vi "AlliGator Image Histogram Panel.vi"() -> ()   [LabVIEW 2021, in "AlliGator Image Histogram.lvlib"]
uses:
  AlliGator Image Histogram.lvlib
  Histograms/Linear Histogram Options.ctl
  Histograms/Histogram Bin Option.ctl
  Histograms/Histogram Bin Position.ctl
  AlliGator Image Histogram Control Refnums.ctl
  Globals, Variables, Constants/AlliGator Refnums List.ctl
  Settings/AlliGator Settings List.ctl
  Action Engine/AlliGator Q Element.ctl
  Action Engine/AlliGator Q Event.ctl
  Source Image/AlliGator Dataset Ctrl Refnums.ctl
  Utilities/Read-Write.ctl
  Graphs/XY Graph/XY Graph Event.ctl
  <vilib>/Utility/miscctls.llb/LVPoint32TypeDef.ctl
  Variant/Variant to Data/Variant to Boolean.vi
  Settings/AlliGator Settings+.lvlib
  Variant/Variant to Data/Variant to Data.lvlib
  Notebook/Notebook.lvlib
  Action Engine/AlliGator Action Engine.lvlib
  Graphs/XY Graph/XY Graph Add-Ons.lvlib
  Python Plugins API/AlliGator Python Plugins.lvlib
  GUI/AlliGator GUI.lvlib
  Utilities/Utilities.lvlib
  GUI/GUI.lvlib
  Error/Error.lvlib
  Histograms/Histograms.lvlib
panel:
  in  "Pin Button":bool=TRUE
  in  "Histogram Lower Percentile":dbl=1.0 caption="Lower Percentile" min=0.0 max=100.0 format="%#.3f"
  in  "Histogram Upper Percentile":dbl=1.0 caption="100 - Upper Percentile" min=0.0 max=100.0 format="%#.3f"
  in  "Auto-Adjust Contrast":bool=TRUE
  in  "Image Histogram Active":bool=TRUE
  in  "Use Image Histogram for Contrast":bool=TRUE
  out "Image Histogram":cluster{"X Array":dbl[], "Y Array":dbl[]}[](graph)
  in  "Image Histogram Options":T1={"Bin Size"=1.0, "Bin Number"=256, "Bin Option"=enum."Bin Number", "Min Value"=-inf, "Max Value"=inf, "Filter NaN & Infinite Values"=TRUE, "Frequency Plot"=FALSE, "Align Bins"=TRUE, "Bin Location"=enum."Left", "Project Outside Values"=FALSE, "Max Histogram Size"=1000000} {"Max Histogram Size" format="%.0e"}
  out "Lower Percentile":dbl=nan format="%#_5g"
  out "Upper Percentile":dbl=nan format="%#_5g"
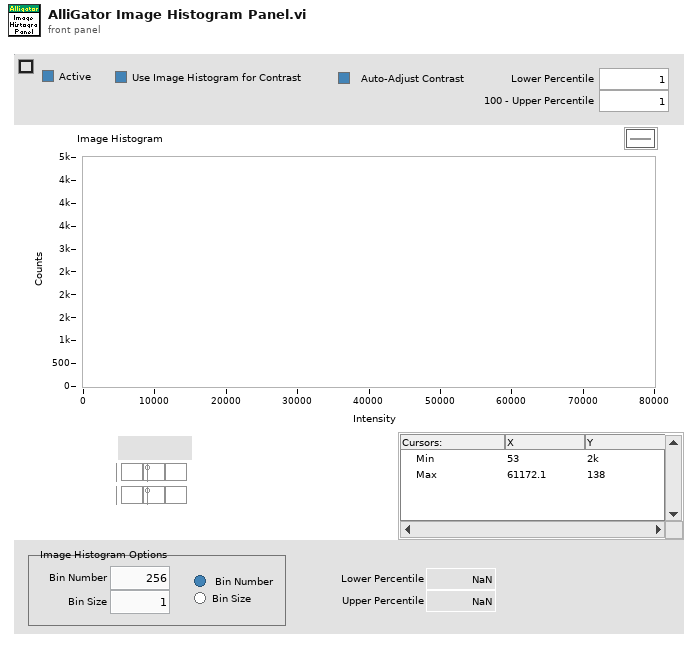
[diagram p1: front panel]
types:
  T1 = typedef "Histograms.lvlib/Linear Histogram Options.ctl" = cluster{"Bin Size":dbl, "Bin Number":i32, "Bin Option":T2, "Min Value":dbl, "Max Value":dbl, "Filter NaN & Infinite Values":bool, "Frequency Plot":bool, "Align Bins":bool, "Bin Location":T3, "Project Outside Values":bool, "Max Histogram Size":i32}
  T2 = typedef "Histograms.lvlib/Histogram Bin Option.ctl" = enum32{"Bin Number", "Bin Size"}
  T3 = typedef "Histograms.lvlib/Histogram Bin Position.ctl" = enum16{"Left", "Center", "Right"}
  T4 = typedef "AlliGator GUI.lvlib/AlliGator Refnums List.ctl" = enum16{"---------- AlliGator Control Refnums ----------", "AlliGator Tab Control Refnum", "Dataset Ctrl Refnums", "Image Histogram Ctrl Refnums", "Intensity Time Trace Ctrl Refnums", "Decay Graph Ctrl Refnums", "Decay Statistics Graph Ctrl Refnums", "Phasor Graph Ctrl Refnums", "Phasor Ratio Graph Ctrl Refnums", "Phasor Plot Ctrl Refnums", "Lifetime & Other Parameters Ctrl Refnums", "Decay Fit Parameter Map Ctrl Refnums", "Parameter Map Ctrl Refnums", "Other AlliGator Ctrl Refnums", "---------- AlliGator Menu Refnums ----------", "AlliGator Menu", "---------- IO Device ID ----------", "Mouse ID", "Keyboard ID"}
  T5 = typedef "AlliGator Image Histogram.lvlib/AlliGator Image Histogram Control Refnums.ctl" = cluster{"Image Histogram":refnum<vi>, "Image Histogram Options":refnum<vi>, "Image Histogram Active":refnum<vi>, "Image Histogram Upper Percentile":refnum<vi>, "Image Histogram Lower Percentile":refnum<vi>, "Auto-Adjust Contrast":refnum<vi>}
  T6 = typedef "AlliGator Settings+.lvlib/AlliGator Settings List.ctl" = enum16{"GUI:Visible Settings Tab", "GUI:Last Run Version", "Source Image:Use Image Histogram for Contrast", "Source Image:Low Count Pixels Rejection Options", "Source Image:High Count Pixels Rejection Options", "Source Image:Use Image Brightness", "Source Image:Blend Overlay with Image Background", "Source Image:Use Fixed ROI Diameter", "Source Image:ROI Diameter", "Source Image:ROI Center Color", "Source Image:Peak Threshold", "Source Image:Intensity Threshold", "Source Image:Image Binning Options", "Source Image:Image Smoothing Options", "Source Image:Image Histogram Active", "Source Image:Invert Binary Mask", "Source Image:Hot Pixel Removal", "Source Image:Overlay Analyzed ROI Center", "Source Image:Auto-Adjust Contrast", "Source Image:Histogram Lower Percentile", "Source Image:Histogram Upper Percentile", "Source Image:Lock ROI with Maps", "Source Image:Save Source Image", "Source Image:Scale Bar Options", "Source Image:Image Resolution (Pixel Size)", "Source Image:Flatfield Correction", "Source Image:Show Dead Left Columns Correction", "Source Image:Dead Left Columns Correction", "Source Image:Image Pre-Processing Operations Order", "Source Image:Overlay ROI Median", "Source Image:Median Overlay Color", "Data Information:Gate Width", "Data Information:Nanotime Gate Separation", "Data Information:Macrotime Gate Separation", "Data Information:Gate Step", "Data Information:# Gates", "Data Information:Gate Image Exposure", "Data Information:Gate Image Integration", "Data Information:Gates to Skip", "Data Information:Gates to Keep", "Data Information:Define Gates to", "Data Information:Channel Name", "Data Information:Available Channel Names", "Data Information:Channel Arithmetic", "Data Information:Background File Subtraction", "Data Information:Background File", "Data Information:Background Scaling Factor", "Data Information:Background Pile-up Correction", "Data Information:Background Pixel Well Capacity", "Data Information:Laser Period", "Data Information:SYNC Period", "Data Information:Pile-up Correction", "Data Information:Pixel Well Capacity", "Data Information:Dataset Scaling Factor", "Fluorescence Decay_Decay Pre-Processing:Reverse Gates", "Fluorescence Decay_Decay Pre-Processing:Verbose Decay Pre-Processing", "Fluorescence Decay_Decay Pre-Processing:Use Decay Pre-Processing", "Fluorescence Decay_Decay Pre-Processing:Background Subtraction", "Fluorescence Decay_Decay Pre-Processing:Background Definition Range", "Fluorescence Decay_Decay Pre-Processing:Baseline Subtraction Method", "Fluorescence Decay_Decay Pre-Processing:Decay Pre-Processing Operations Order", "Fluorescence Decay_Decay Pre-Processing:Smoothing Parameter", "Fluorescence Decay_Decay Pre-Processing:Shift Decay", "Fluorescence Decay_Decay Pre-Processing:Decay Shift Parameters", "Fluorescence Decay_Decay Pre-Processing:Fold Decay", "Fluorescence Decay_Decay Pre-Processing:# Folds", "Fluorescence Decay_Decay Pre-Processing:1-Normalize Decay", "Fluorescence Decay_Decay Pre-Processing:[0-1]-Normalize Decay", "Fluorescence Decay_Decay Pre-Processing:Smoothen Decay", "Fluorescence Decay_Decay Pre-Processing:Extrapolate Decay", "Fluorescence Decay_Decay Pre-Processing:Use Periodicity", "Fluorescence Decay_Decay Pre-Processing:Use Cursors", "Fluorescence Decay_Decay Pre-Processing:Tail Fraction", "Fluorescence Decay_Decay Pre-Processing:Head Fraction", "Fluorescence Decay_Decay Pre-Processing:Additional Points", "Fluorescence Decay_Decay Pre-Processing:Straighten Decay", "Fluorescence Decay_Decay Pre-Processing:Constant Background", "Fluorescence Decay_Decay Pre-Processing:Pixel-Normalize Decay", "Fluorescence Decay_Advanced Analysis:Extract IRF instead of Decay", "Fluorescence Decay_Advanced Analysis:IRF Extraction Options", "Fluorescence Decay_Advanced Analysis:IRF Optimization Options", "Fluorescence Decay_Advanced Analysis:Square Pulse Options", "Fluorescence Decay_Advanced Analysis:IRF Order", "Fluorescence Decay_Advanced Analysis:IRF Time Constants", "Fluorescence Decay_Advanced Analysis:Wavelet Analysis Options", "Fluorescence Decay_Advanced Analysis:Average Lifetime Options", "Fluorescence Decay_Fit Options:Fit Options", "Fluorescence Decay_Fit Options:Use Legacy Fitting Approach", "Fluorescence Decay_Fit Options:Use Data Information Laser Period", "Fluorescence Decay_Fit Parameters:Displayed Fit Parameters", "Fluorescence Decay_Fit Parameters:Fit Parameter Constraints", "Fluorescence Decay_Fit Parameters:Export Tabulated Results", "Fluorescence Decay_Fit Parameters:MLE Baseline Offset Type", "Fluorescence Decay_Fit Parameters:MLE Baseline Offset", "Fluorescence Decay_Fit Parameters:Guess Parameter Names", "Fluorescence Decay_Fit Parameters:Guess Parameter Values", "Fluorescence Decay_Fit Parameters:Guess Parameters Options", "Fluorescence Decay_Fit Parameters:Optimal Offset Selection Criterion", "Fluorescence Decay_Styles:Show Last Decay Only", "Fluorescence Decay_Styles:Decay Graph Color Array", "Fluorescence Decay:Decay Graph Active", "Fluorescence Decay Statistics:Min Peak Value", "Fluorescence Decay Statistics:Reject Low Decay Peak Pixels", "Fluorescence Decay Statistics:Reject High Decay Peak Pixels", "Fluorescence Decay Statistics:Max Peak Value", "Time Traces:Use File Timestamp", "Time Traces:Time Step", "Time Traces:Use Intensity Correction File", "Time Traces:Intensity Correction File", "Phasor Plot:Phasor Plot Smoothing Options", "Phasor Plot:Phasor Plot Size", "Phasor Plot:Phasor Plot Graphics Options", "Phasor Plot:Cumulative Phasor Plot", "Phasor Plot:Use Phasor Brightness", "Phasor Plot:Blend Overlay with Phasor Background", "Phasor Plot:Save Phasor Plot", "Phasor Plot:Show References", "Phasor Plot:Phasor Ratio Decay Range", "Phasor Plot:Exponential Fading", "Phasor Plot:Phasor Ratio Reference Colors", "Phasor Plot:Reference Radius", "Phasor Plot:Show Color Map Vertices", "Phasor Plot:Phasor Plot Active", "Phasor Plot:Phasor Ratio Color Map Type", "Phasor Plot:Phasor Ratio Color Map", "Phasor Plot:Phasor Ratio Display Range", "Phasor Plot:Selected Image ROI(s)", "Phasor Plot:All Image ROIs", "Phasor Plot:Selected Phasor Plot ROI(s)", "Phasor Plot:All Phasor Plot ROIs", "Phasor Plot:Phasor Ratio Color-Coded Quantity", "Phasor Plot:Store Phasor Harmonics", "Phasor Plot:Draw Reference Segment", "Phasor Plot:User-Defined Quantity", "Phasor Plot:Color Scale High Color", "Phasor Plot:Color Scale Low Color", "Phasor Plot:Intensity-weighted Phasor Plot", "Phasor Graph:Phasor Frequency", "Phasor Graph:Phasor Ratio Type", "Phasor Graph:Pixel-level Phasor Computation", "Phasor Graph:Save Phasor Graph", "Phasor Graph:Phasor Graph Active", "Phasor Graph:Phasor SDV Options", "Phasor Graph:Intensity-weighted Phasor Graph", "Phasor Graph:Define Shortest Lifetime as", "Phasor Calibration:Use Backup Calibration if needed", "Phasor Calibration:Backup Calibration Type", "Phasor Calibration:Calibration Type", "Phasor Calibration:Calibration Lifetime", "Phasor Calibration:Calibration Map Algorithm", "Single-Exponential Phasor Locus (SEPL):Gate Parameters", "Single-Exponential Phasor Locus (SEPL):User-defined Gate", "Single-Exponential Phasor Locus (SEPL):User-defined IRF", "Single-Exponential Phasor Locus (SEPL):Phasor Parameters", "Single-Exponential Phasor Locus (SEPL):Decay & IRF Parameters", "Single-Exponential Phasor Locus (SEPL):Display Parameters", "Lifetime Analysis:Decay Analysis Parameters", "Lifetime Analysis:Lifetime Map Active", "Plugins:Python Settings", "Miscellaneous:Verbose Mode", "Miscellaneous:Beep after Script", "Miscellaneous:Saved Image File Format", "Miscellaneous:Exported Gate Image Settings", "Miscellaneous:Include Loading in Timing", "Miscellaneous:Verbose Settings Mode", "Miscellaneous:Histogram Options", "Miscellaneous:Beep on Error", "Miscellaneous:# Logical Processors Used", "Miscellaneous:ROI Description Max Characters", "Miscellaneous:Verbose Error Mode", "Miscellaneous:Transparent Mask Color"}
  T7 = typedef "AlliGator Action Engine.lvlib/AlliGator Q Element.ctl" = cluster{"AlliGator Q Event":T8, "Data":variant}
  T8 = typedef "AlliGator Action Engine.lvlib/AlliGator Q Event.ctl" = enum16{"---- Files ----", "Files:Set Batch Export Files To Save", "Files:Set Dataset Loading & Pre-processing Options", "Files:Check #Frames in Dataset", "Files:Increment Frame Index", "Files:Open Mask Image", "Files:Open White Light Image", "Files:Open Single Dataset", "Files:New Folder of Folders Selected", "Files:Load File (all Types)_Scriptable", "Files:Move Flattened Series to Folders Series", "Files:Select Folder", "Files:Load FLI Dataset", "Files:Load Swiss SPAD 1 Dataset", "Files:Load Swiss SPAD 2 Dataset", "Files:Load .sdt FLI Dataset", "Files:Load .ptu FLI Dataset", "Files:Load .bin FLI Dataset", "Files:Load Single Gate Image Folder", "Files:Load I/m/phi Dataset (deprecated)", "Files:Load Single Image", "Files:Subtract Background File", "Files:Export FLI Dataset", "Files:Load HDF5 FLI Dataset", "Files:Set Destination File Path", "Files:Save Mask Image", "Files:Batch Conversion", "Files:New Folder Selected", "Files:Close FLI Dataset", "Files:Close FLI Dataset Series", "Files:Close White Light Image", "Files:Close Mask Image", "---- FLI Dataset ----", "FLI Dataset:Channel Arithmetic", "FLI Dataset:Export Average Lifetime Map as ASCII", "FLI Dataset:Export User-Defined Quantity Map as ASCII", "FLI Dataset:Python Function FLI Dataset Event", "FLI Dataset:ROI Analysis", "FLI Dataset:Tilted Logistic Square Gated IRF Characteristics Map", "FLI Dataset:Logistic Square Gated IRF Characteristics Map", "FLI Dataset:Square Gated IRF Characteristics Map", "FLI Dataset:Multi-ROI Single-Pixel Phasor Analysis", "FLI Dataset:Multi-ROI Single-Pixel NLSF Analysis", "FLI Dataset:All ROIs IRF Extraction", "FLI Dataset:All ROIs Decay Fit Non-Interactive (Fast + Individual IRF)", "FLI Dataset:All ROIs Phasor Analysis", "FLI Dataset:All ROIs Decay Fit", "FLI Dataset:Fluorescence Decay Statistics", "FLI Dataset:Update Decay Statistics Graph", "FLI Dataset:Get Decay from ROI", "FLI Dataset:All ROIs Average Lifetimes", "FLI Dataset:Save/Load Local IRFs", "FLI Dataset:Clear Local IRFs", "FLI Dataset:Phasor Calibration Maps (# Gates Series) Script", "FLI Dataset:Calibrated Phasor Map Series", "---- FLI Dataset Series ----", "FLI Dataset Series:Sum All Datasets in Series", "FLI Dataset Series:Add Dataset to Accumulated Dataset", "FLI Dataset Series:Display Accumulated Dataset", "FLI Dataset Series:Clear Dataset Series Sum", "FLI Dataset Series:Time-Series Analysis (NLSF)", "FLI Dataset Series:Time-Series Analysis (Phasor)", "---- Image ----", "Image:Update Image Profile Plots", "Image:Image Histogram Cursor Move", "Image:Image Histogram", "Image:Image Contrast", "Image:Set Image Histogram Cursor Move Flag", "Image:Clear Image Overlay", "Image:Use ROI as Search Area", "Image:Set ROI Diameter", "Image:Save Image Data as TIFF", "Image:Save Displayed Image with Overlay", "Image:Save Image Overlay Only", "Image:Save Image as Hot Pixel Mask", "Image:Change Source Image Color Palette", "Image:Copy Image to Clipboard", "Image:Source Image ROI Selection", "Image:Delete All ROIs", "Image:Delete All Unselected ROIs", "Image:Delete ROI", "Image:Merge All ROIs", "Image:Store ROI", "Image:Source Image ROI Storage", "Image:Export ROI Description to Notebook", "Image:Save ROI", "Image:Load ROI", "Image:Paste ROI Definition", "Image:Clear ROI", "Image:Identify ROIs in Mask Image", "Image:Create Complementary ROI", "Image:Create Contour ROI", "Image:Create ROI(s) from Pixels with Peak above Min_Scriptable", "Image:Create ROI(s) from Pixels with Intensity above Min_Scriptable", "Image:Compute ROI Statistics", "Image:Delete ROI(s) based on ROI Characteristics", "Image:Create ROI Grid", "Image:ROI to Individual Pixel ROIs", "Image:Python Function Source Image Event", "Image:Show Phasor Calibration Map ROI Centers", "Image:Convert ROI to Mask Image", "Image:Mouse Move", "Image:Mouse Up", "Image:Set Source Image Mouse Move Flag", "Image:Add Scale Bar Overlay", "Image:Delete Existing ROIs Option", "Image:Overlay ROI Median", "Image:Check Current ROI", "Image:Update True Pixel Value", "Image:Use ROI", "---- Decay ----", "Decay:Clear IRF/Reference Plot", "Decay:Add Decay to Graph", "Decay:Smoothen Plot", "Decay:Smoothen Plot Tail", "Decay:Average Selected Plots", "Decay:Extract IRF", "Decay:Optimal IRF Extraction", "Decay:Threshold IRF", "Decay:Fit to Model IRF", "Decay:Fit IRF to Square Gate", "Decay:Fit IRF to Logistic Square Gate", "Decay:Fit IRF to Tilted Logistic Square Gate", "Decay:Create Bounding Cursors Set", "Decay:Export Bounding Cursors Definition to Notebook", "Decay:Denoise Plot", "Decay:Compute Cumulative Function", "Decay:Use as Reference Decay", "Decay:Show Reference Decay/IRF", "Decay:Extrapolate Decay", "Decay:Create Head & Tail Bounding Cursors", "Decay:Store Cursor-defined Head & Tail Fractions", "Decay:Rebin Plot", "Decay:1-Normalize Decay", "Decay:[0-1]-Normalize Plot", "Decay:Straighten Decay", "Decay:Shift Decay", "Decay:Fold Decay", "Decay:Fit Decay", "Decay:Global Fit of Selected Decays", "Decay:Post Global Fit Script", "Decay:Add Global Fit Parameters to Graph", "Decay:Add Decay Parameter(s) to Plot (Graph)", "Decay:Export Decay to Phasor Graph", "Decay:Compute Average Lifetime", "Decay:Plot Convolution", "Decay:Graph Tip Strip Update", "---- Decay Statistics ----", "Decay Statistics:Tip Strip Update", "---- Intensity Time Trace ----", "Intensity Time Trace:Use File Timestamp", "Intensity Time Trace:Load Intensity Corrections File", "Intensity Time Trace:Clear Intensity Corrections File", "Intensity Time Trace:Tip Strip Update", "---- Phasor Plot ----", "Phasor Plot:Build Phasor Plot", "Phasor Plot:Change Phasor Plot Color Palette", "Phasor Plot:Adjust Phasor Plot Display Range", "Phasor Plot:Highlight Image ROI in Phasor Plot", "Phasor Plot:Save Phasor Plot Image with Overlay", "Phasor Plot:Export Complex Phasor Map", "Phasor Plot:Export Phasor Ratio Map", "Phasor Plot:Export Average Lifetime Map", "Phasor Plot:Compute Phase Lifetime Histogram", "Phasor Plot:Compute Phasor Ratio Histogram", "Phasor Plot:Compute Phase Lifetime vs Intensity Scatter Plot", "Phasor Plot:Weber 2-Component Decomposition", "Phasor Plot:Update Phasor Color Map Vertices", "Phasor Plot:Clear Phasor Overlay", "Phasor Plot:Use Segment Extremities as References", "Phasor Plot:Use UC/Segment Intersections as References", "Phasor Plot:Use UC/Principal Axis Intersections as References", "Phasor Plot:Use UC/Linear Fit Intersections as References", "Phasor Plot:Update Phasor Plot Reference", "Phasor Plot:Show Local Phasor Info in Phasor Plot", "Phasor Plot:Update Phasor Plot State", "Phasor Plot:Phasor Plot ROI Storage", "Phasor Plot:Phasor Plot ROI Selection", "Phasor Plot:Python Function Phasor Plot Event", "Phasor Plot:Overlay Phasor ROI, Ratio or Map in Source Image", "Phasor Plot:Compute Decay of Selected Phasors", "Phasor Plot:Phasor at Image Pixel", "Phasor Plot:Mouse Move", "Phasor Plot:Mouse Up", "Phasor Plot:Display Range Mouse Move", "Phasor Plot:Set Mouse Move Flag", "Phasor Plot:Update True Phasor Plot Value", "---- Phasor Graph ----", "Phasor Graph:Get Phasor Value", "Phasor Graph:Create New Phasor Plot Dialog", "Phasor Graph:Update Last Phasor Value", "Phasor Graph:Update Phasor (m, phi)", "Phasor Graph:Remove Single Phasor from Plot", "Phasor Graph:Add Single Phasor to Plot", "Phasor Graph:Remove Phasor Plot", "Phasor Graph:Remove Selected Phasor Plots", "Phasor Graph:Clear Phasor Data", "Phasor Graph:Clear Phasor Graph", "Phasor Graph:Cursor Move", "Phasor Graph:Draw Cursor Connecting Line", "Phasor Graph:Clear Cursor Connecting Line", "Phasor Graph:Find UC Intersection", "Phasor Graph:Use UC/Cursor-Defined Line Intersections", "Phasor Graph:Use Selected Plots Fitted Line/UC Intersections", "Phasor Graph:Use Selected Plots Principal Axis/UC Intersections", "Phasor Graph:Show Single Phasor", "Phasor Graph:Save Single Phasor Plot", "Phasor Graph:Save All Phasor Plots", "Phasor Graph:Load Phasor Plot(s)", "Phasor Graph:Phasor Multiplication", "Phasor Graph:Compute Average Phasor", "Phasor Graph:Compute Multiple Average Phasors (Selected Plots)", "Phasor Graph:Export Single Phasor Plot Phase Lifetimes", "Phasor Graph:Parameter 2 vs Parameter 1 Scatter Plot", "Phasor Graph:Use Cursor n Location", "Phasor Graph:Set Reference n to Current Phase Lifetime Value", "Phasor Graph:Set Reference n to Lifetime Value", "Phasor Graph:Set Cursor n Location", "Phasor Graph:Save Phasor Graph Image", "Phasor Graph:Update SEPL Plot", "Phasor Graph:Export Single Phasor Plot Data", "Phasor Graph:Export Selected Phasor Plots Data", "Phasor Graph:Python Function Phasor Graph Event", "Phasor Graph:Tip Strip Update", "---- Calibration ----", "Calibration:Set Calibration Type", "Calibration:Load/Save Phasor Calibration", "Calibration:Load/Save Phasor Calibration Series", "Calibration:Load/Save Phasor Calibration Map", "Calibration:Use as Calibration", "Calibration:Compute Optimal Calibration from Phasor References", "Calibration:Clear Phasor Calibration", "Calibration:Single Phasor Calibration Information", "Calibration:Use as Calibration Series", "Calibration:Use as Calibration Map", "Calibration:Clear Calibration Series", "Calibration:Phasor Calibration Series Information", "Calibration:Clear Calibration Map", "Calibration:Phasor Calibration Map Information", "Calibration:Apply Phasor Calibration", "Calibration:Update Single Plot Calibration", "Calibration:Update Multiple Plots Calibration", "Calibration:Clear Single Plot Calibration", "Calibration:Clear All Plots Calibrations", "Calibration:Clear Plot(s) Calibration(s)?", "---- Phasor Ratio ----", "Phasor Ratio:Clear Reference n", "Phasor Ratio:Toggle Selected Plot(s)  Lock to Reference 1", "Phasor Ratio:Use as Reference n", "Phasor Ratio:Send Reference n to Notebook", "Phasor Ratio:Toggle Selected Plot(s)  Lock to Reference 2", "Phasor Ratio:Compute Phasor Ratio at Mouse Location", "Phasor Ratio:Compute Phasor Plot's Average Phasor Ratio", "Phasor Ratio:Compute Time-Series Phasor Ratios", "Phasor Ratio:Fit Line to Phasor Ratio Plot", "Phasor Ratio:Save References", "Phasor Ratio:Load References", "Phasor Ratio:Update Phasor Reference 1", "Phasor Ratio:Update Phasor Reference 2", "Phasor Ratio:Move Cursor n to Reference n", "Phasor Ratio:Use as Phasor Reference 1 Lifetime", "Phasor Ratio:Use as Phasor Reference 2 Lifetime", "Phasor Ratio:Export Phasor Ratio Map as ASCII", "Phasor Ratio:Tip Strip Update", "---- Lifetime & Other Parameters Graph ----", "Lifetime:Compute Sliced Mean, SDV and CV Plots", "Lifetime:Plot Decay Shifts", "Lifetime:Plot Histogram", "---- Decay Fit Parameter Map ----", "Decay Fit Parameter Map:Export ROI NLSF Data as ASCII", "Decay Fit Parameter Map:Set Decay Fit Parameter Map Selection", "Decay Fit Parameter Map:Build Decay Fit Parameter Map", "Decay Fit Parameter Map:Change Decay Fit Parameter Map Color Palette", "Decay Fit Parameter Map:Export Decay Fit Parameter Map Data as ASCII", "Decay Fit Parameter Map:Export All Decay Fit Parameter Maps Data as ASCII", "Decay Fit Parameter Map:Selected Parameter Scatterplot", "Decay Fit Parameter Map:Parameter 2 vs Parameter 1 Scatterplot", "Decay Fit Parameter Map:Save Decay Fit Parameter Map Image", "Decay Fit Parameter Map:Save-Load IRFs & Fit Data", "Decay Fit Parameter Map:Update Local Decay Plots", "Decay Fit Parameter Map:Python Function Decay Fit Parameters Map Event", "Decay Fit Parameter Map:Overlay Decay Fit Parameter Map in Source Image", "Decay Fit Parameter Map:Selected Parameter vs Intensity Scatterplot", "Decay Fit Parameter Map:Mouse Up", "Decay Fit Parameter Map:Mouse Move", "Decay Fit Parameter Map:Display Range Mouse Move", "Decay Fit Parameter Map:Change Map Resolution", "Decay Fit Parameter Map:Variance Significance Maps", "Decay Fit Parameter Map:Fit Result Constraints Window", "Decay Fit Parameter Map:Use ROI", "---- Parameter Map ----", "Parameter Map:Export ROI Parameters Data as ASCII", "Parameter Map:Add Parameter Map Set", "Parameter Map:Delete Parameter Map Set", "Parameter Map:Update Parameter List", "Parameter Map:Build Parameter Map", "Parameter Map:Change Parameter Map Color Palette", "Parameter Map:Export Parameter Map Data as ASCII", "Parameter Map:Export All Parameter Maps Data as ASCII", "Parameter Map:Selected Parameter Scatterplot", "Parameter Map:Parameter 2 vs Parameter 1 Scatterplot", "Parameter Map:Selected Parameter vs Intensity Scatterplot", "Parameter Map:Save Parameter Map Image", "Parameter Map:Save-Load IRFs & Parameter Maps (TODO)", "Parameter Map:Set Parameter Map Selection", "Parameter Map:Python Function Parameter Map Event", "Parameter Map:Overlay Parameter Map in Source Image", "Parameter Map:Update Local Decay Plots", "Parameter Map:Mouse Up", "Parameter Map:Mouse Move", "Parameter Map:Display Range Mouse Move", "Parameter Map:Use ROI", "---- Generic Graph ----", "Generic Graph:Generic XY Graph Event", "Generic Graph:Python Function XY Graph Event", "Generic Graph:New Plot", "Generic Graph:Save Plot", "Generic Graph:XY Plot Histogram", "Generic Graph:Set XY Graph Plot Name", "Generic Graph:Set Last Cursor Style", "Generic Graph:Tip Strip Update", "---- GUI ----", "GUI:Start Script", "GUI:Type of Displayed Image Changed", "GUI:Gate Image Slide Changed", "GUI:Show Busy Icon", "GUI:Show Busy Icon & Abort Button", "GUI:Hide Busy Icon", "GUI:Hide Busy Icon & Abort Button", "GUI:Abort", "GUI:End Script", "GUI:Start Timing", "GUI:End Timing", "GUI:Set State Indicator", "GUI:Send Parameters JSON Strings to Clipboard", "GUI:Set Gate Step", "GUI:Idle", "GUI:Initialization", "GUI:Quit", "GUI:Increment Dataset Index", "GUI:Set Dataset Index to -1", "GUI:Time Series Slider Moved", "GUI:Time Series Slider Changed", "GUI:Toggle Playback or Loop", "GUI:Playback Script", "GUI:Set Phasor Frequency", "GUI:Open Window", "GUI:Start Test Script", "GUI:End Test Script", "GUI:Set Verbose Mode", "GUI:Set Verbose Settings Mode", "GUI:Initialize Python Session", "DEBUG"}
  T9 = typedef "Utilities.lvlib/Read-Write.ctl" = enum16{"Read", "Write"}
  T10 = typedef "AlliGator GUI.lvlib/AlliGator Dataset Ctrl Refnums.ctl" = cluster{"Current Data":refnum<vi>, "Gate Image Slide":refnum<vi>, "Time Point Slide":refnum<vi>, "Current Time Stamp":refnum<vi>, "Save Image":refnum<vi>, "Displayed Image":refnum<vi>, "Phasor Overlay Color":refnum<vi>, "Image Color Scale":refnum<vi>, "Use ROI as Search Area":refnum<vi>, "Source Image ROI Color":refnum<vi>, "True Pixel Value":refnum<vi>, "Source Image Display":refnum<vi>, "CPU":refnum<vi>}
  T11 = enum16{"0", "1", "2", "3", "4", "5", "6", "7", "8", "9", "A", "B", "C", "D", "E", "F", "G", "H", "I", "J", "K", "L", "M", "N", "O", "P", "Q", "R", "S", "T", "U", "V", "W", "X", "Y", "Z", "F1", "F2", "F3", "F4", "F5", "F6", "F7", "F8", "F9", "F10", "F11", "F12", "F13", "F14", "F15", "ADD", "BACK", "BACKSLASH", "CAPITAL", "COMMA", "DECIMAL", "DELETE", "DIVIDE", "DOWN", "END", "EQUALS", "ESCAPE", "GRAVE (`)", "HOME", "INSERT", "LBRACKET", "LCONTROL", "LEFT", "L ALT", "LSHIFT", "LWIN", "MINUS", "MULTIPLY", "NEXT", "NUMLOCK", "NUMPAD_0", "NUMPAD_1", "NUMPAD_2", "NUMPAD_3", "NUMPAD_4", "NUMPAD_5", "NUMPAD_6", "NUMPAD_7", "NUMPAD_8", "NUMPAD_9", "PAUSE", "PERIOD", "PRIOR (PG UP)", "RBRACKET", "RCONTROL", "RETURN", "RIGHT", "R ALT", "RSHIFT", "RWIN", "SCROLL", "SEMICOLON", "SLASH", "SPACE", "SUBTRACT", "TAB", "UP", "ENTER (num pad)", "' (quote)"}
  T12 = typedef "XY Graph Add-Ons.lvlib/XY Graph Event.ctl" = cluster{"Item Tag":string, "XY Graph Refnum":refnum<vi>, "Coords":T13, "Item Path":string}
  T13 = typedef "LVPoint32TypeDef.ctl" = cluster{"Horizontal":i32, "Vertical":i32}
  T14 = typedef "XY Graph Add-Ons.lvlib/XY Graph Refnum.ctl" = refnum<vi>
  T15 = enum16{"0", "1", "2", "3", "4", "5", "6", "7", "8", "9", "A", "B", "C", "D", "E", "F", "G", "H", "I", "J", "K", "L", "M", "N", "O", "P", "Q", "R", "S", "T", "U", "V", "W", "X", "Y", "Z", "F1", "F2", "F3", "F4", "F5", "F6", "F7", "F8", "F9", "F10", "F11", "F12", "F13", "F14", "F15", "ADD", "BACK", "BACKSLASH", "CAPITAL", "COMMA", "DECIMAL", "DELETE", "DIVIDE", "DOWN", "END", "EQUALS", "ESCAPE", "GRAVE (`)", "HOME", "INSERT", "LBRACKET", "LCONTROL", "LEFT", "L ALT", "LSHIFT", "LWIN", "MINUS", "MULTIPLY", "NEXT", "NUMLOCK", "NUMPAD_0", "NUMPAD_1", "NUMPAD_2", "NUMPAD_3", "NUMPAD_4", "NUMPAD_5", "NUMPAD_6", "NUMPAD_7", "NUMPAD_8", "NUMPAD_9", "PAUSE", "PERIOD", "PRIOR (PG UP)", "RBRACKET", "RCONTROL", "RETURN", "RIGHT", "R ALT", "RSHIFT", "RWIN", "SCROLL", "SEMICOLON", "SLASH", "SPACE", "SUBTRACT", "TAB", "UP", "ENTER (num pad)", "' (quote)"}[]
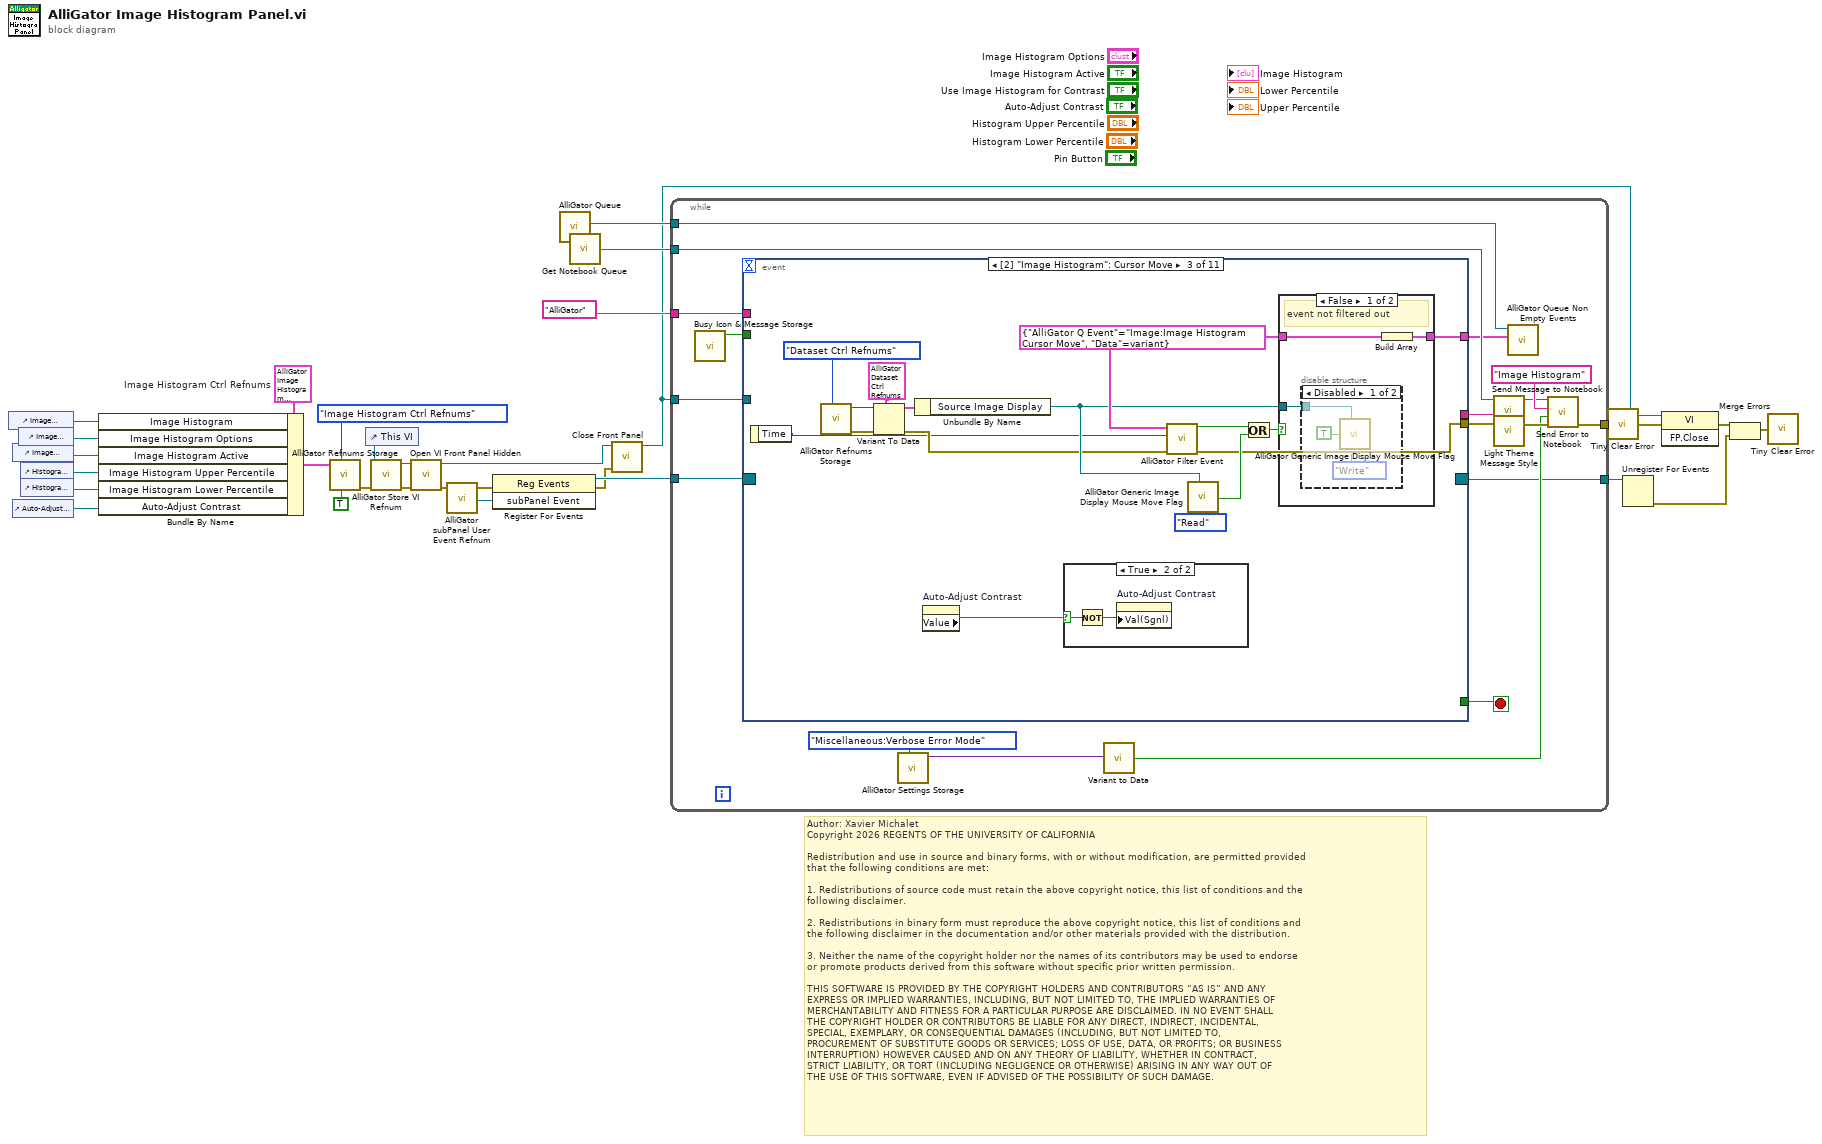
[diagram p0: block diagram]
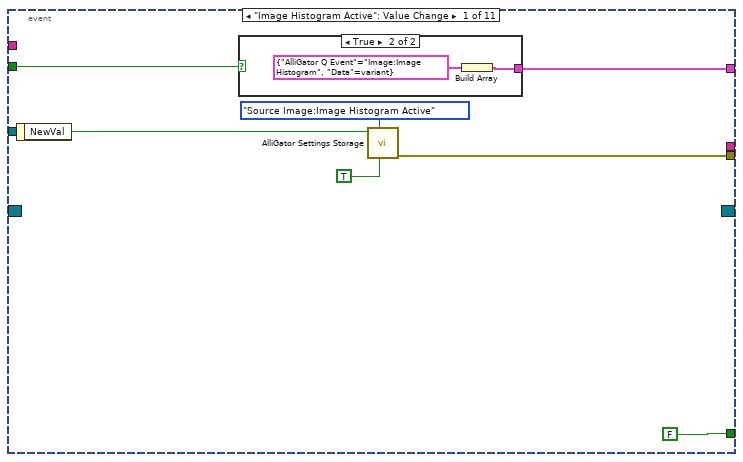
[diagram p2: hidden frame]
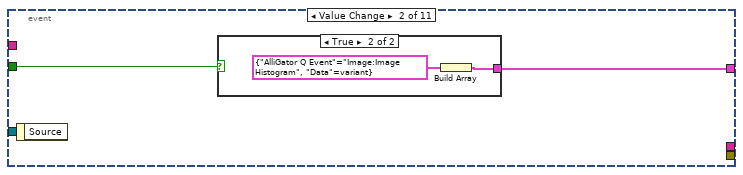
[diagram p4: hidden frame]
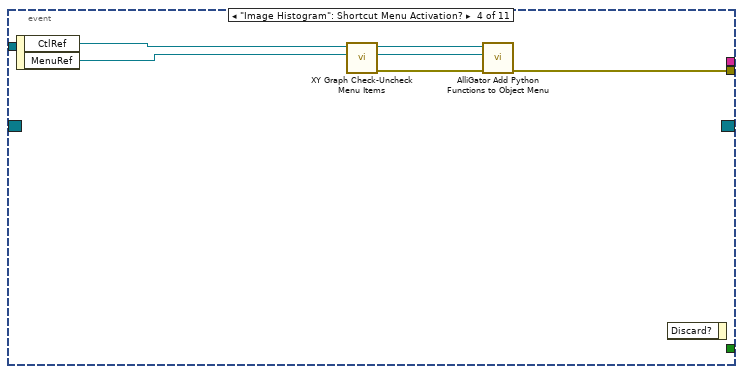
[diagram p9: hidden frame]
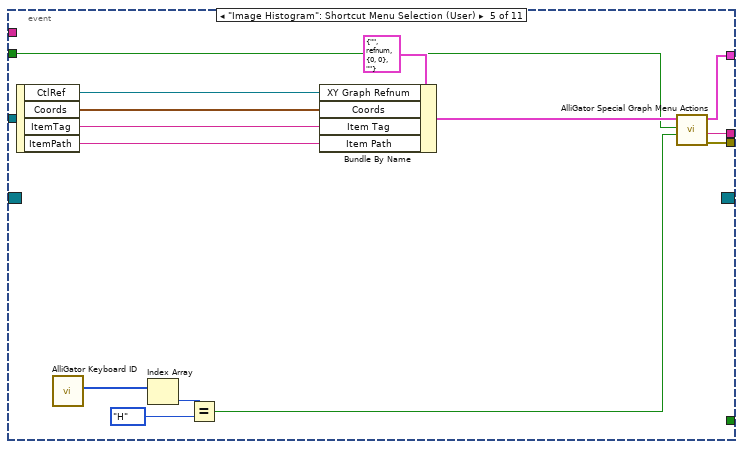
[diagram p10: hidden frame]
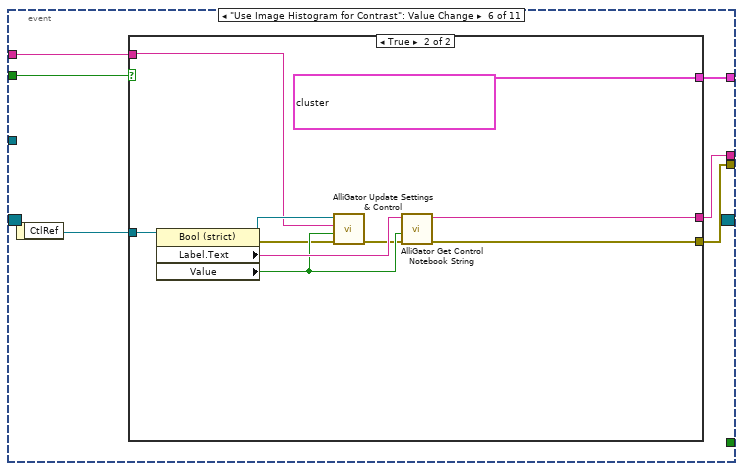
[diagram p11: hidden frame]
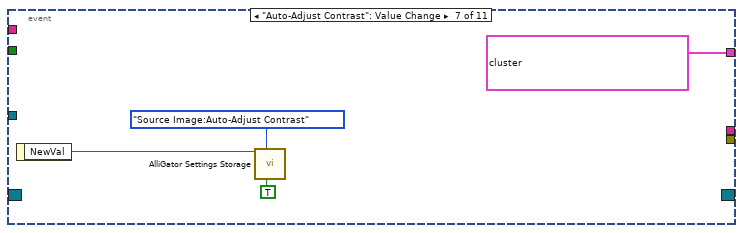
[diagram p13: hidden frame]
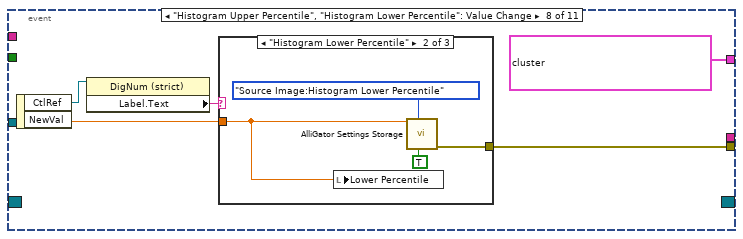
[diagram p14: hidden frame]
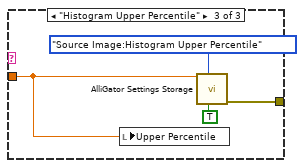
[diagram p16: hidden frame]
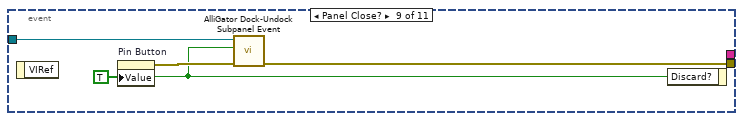
[diagram p17: hidden frame]
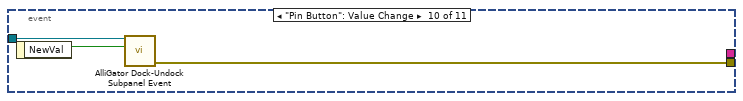
[diagram p18: hidden frame]
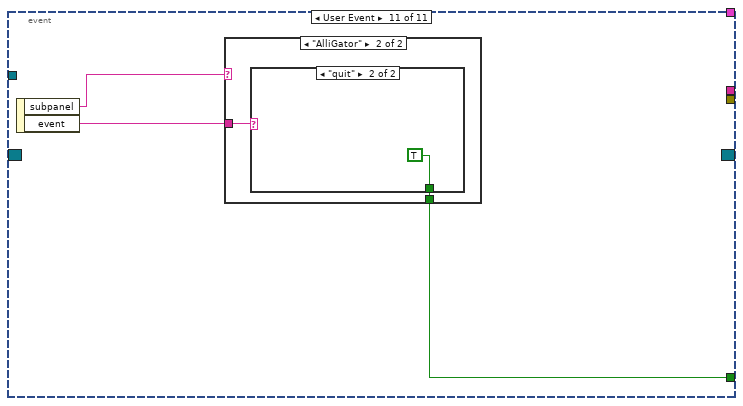
[diagram p19: hidden frame]
diagram:
  w21 = T5 {"Image Histogram"=refnum, "Image Histogram Options"=refnum, "Image Histogram Active"=refnum, "Image Histogram Upper Percentile"=refnum, "Image Histogram Lower Percentile"=refnum, "Auto-Adjust Contrast"=refnum}  # Image Histogram Ctrl Refnums
  # "Author: Xavier Michalet\nCopyright 2026 REGENTS OF THE UNIVERSITY OF CALIFORNIA\n\nRedistribution and use in source and binary forms, with or without modification, are permitted provided\nthat the following conditions are met:\n\n1. Redistributions of source code must retain the above copyright notice, this list of conditions and the\nfollowing disclaimer.\n\n2. Redistributions in binary form must reproduce the above copyright notice, this list of conditions and\nthe following disclaimer in the documentation and/or other materials provided with the distribution.\n\n3. Neither the name of the copyright holder nor the names of its contributors may be used to endorse \nor promote products derived from this software without specific prior written permission.\n\nTHIS SOFTWARE IS PROVIDED BY THE COPYRIGHT HOLDERS AND CONTRIBUTORS “AS IS” AND ANY \nEXPRESS OR IMPLIED WARRANTIES, INCLUDING, BUT NOT LIMITED TO, THE IMPLIED WARRANTIES OF\nMERCHANTABILITY AND FITNESS FOR A PARTICULAR PURPOSE ARE DISCLAIMED. IN NO EVENT SHALL\nTHE COPYRIGHT HOLDER OR CONTRIBUTORS BE LIABLE FOR ANY DIRECT, INDIRECT, INCIDENTAL, \nSPECIAL, EXEMPLARY, OR CONSEQUENTIAL DAMAGES (INCLUDING, BUT NOT LIMITED TO, \nPROCUREMENT OF SUBSTITUTE GOODS OR SERVICES; LOSS OF USE, DATA, OR PROFITS; OR BUSINESS\nINTERRUPTION) HOWEVER CAUSED AND ON ANY THEORY OF LIABILITY, WHETHER IN CONTRACT, \nSTRICT LIABILITY, OR TORT (INCLUDING NEGLIGENCE OR OTHERWISE) ARISING IN ANY WAY OUT OF\nTHE USE OF THIS SOFTWARE, EVEN IF ADVISED OF THE POSSIBILITY OF SUCH DAMAGE."
  n1 = control-ref of="Image Histogram"() -> (w17:refnum<vi>)
  n2 = control-ref of="Image Histogram Active"() -> (w15:refnum<vi>)
  n3 = control-ref of="Auto-Adjust Contrast"() -> (w12:refnum<vi>)
  n4 = control-ref of="Image Histogram Options"() -> (w16:refnum<vi>)
  n5 = control-ref of="Histogram Upper Percentile"() -> (w14:refnum<vi>)
  n6 = control-ref of="Histogram Lower Percentile"() -> (w13:refnum<vi>)
  n7 = Bundle By Name(cluster=w21, "Image Histogram"=w17, "Image Histogram Options"=w16, "Image Histogram Active"=w15, "Image Histogram Upper Percentile"=w14, "Image Histogram Lower Percentile"=w13, "Auto-Adjust Contrast"=w12) -> (w20:T5)
  n8 = call "AlliGator Refnums Storage.vi"("Get(F)/Set"=TRUE, "AlliGator Refnum List"=AlliGator_Refnums_List."Image Histogram Ctrl Refnums", "Data in"=w20) -> ("Error Out"=w4:errorcluster)  [unwired: 7 in, 1 out]
  n9 = control-ref of="This VI"() -> (w2:refnum<vi>)
  n10 = call "AlliGator Store VI Refnum.vi"("error in (no error)"=w4, "VI Refnum"=w2) -> ("error out"=w3:errorcluster, "VI Refnum (dup)"=w1:refnum<vi>)  [unwired: 7 in, 1 out]
  n11 = call "Open VI Front Panel Hidden.vi"("error in"=w3, "VI in"=w1) -> ("error out"=w8:errorcluster, "VI out"=w7:refnum<vi>)  [unwired: 8 in]
  n12 = call "AlliGator subPanel User Event Refnum.vi"() -> ("subPanel Event"=w26:refnum<user-event>)  [unwired: 9 in]
  n13 = register-events(error in=w8, w26) -> (reference out=w25:refnum<event-registration>, error out=w5:errorcluster)  [unwired: 1 in]
  n14 = call "AlliGator Queue.vi"() -> ("AlliGator Q"=w28:refnum<queue>)  [unwired: 8 in, 1 out]
  n15 = call "Get Notebook Queue.vi"() -> ("Notebook Queue"=w29:refnum<queue>)  [unwired: 9 in]
  n16 = call "Close Front Panel.vi"("error in (no error)"=w5, "VI in"=w7) -> ("VI out"=w6:refnum<vi>)  [unwired: 8 in, 1 out]
  n17 = while {
    tunnel: w29 -> [w40]
    tunnel: w28 -> [w37]
    tunnel: "AlliGator" ("Sender") -> [w35]
    tunnel: w6 -> [w33]
    tunnel: w25 -> [w32]
    tunnel: [w31] -> w24
    tunnel: [w30] -> w23
    stop <- w47 stop-if-true
    n18 = call "Busy Icon & Message Storage.vi"() -> ("Busy Icon Status (F = busy)"=w34:bool)  [unwired: 9 in, 2 out]
    n19 = event shown="[2] \"Image Histogram\": Cursor Move" {
      selector: w32 -> [_ _ _ _ _ _ _ _ _ _ _]
      dyn-events: [_ _ _ _ _ _ _ _ _ _ _] -> w31
      timeout: _ -> [_ _ _ _ _ _ _ _ _ _ _]
      tunnel: [w51 _ w64 w85 w98 w108 _ w125 w140 w142 _] -> w41
      tunnel: [FALSE _ _ _ _ _ _ _ _ _ w145] -> w47
      tunnel: [_ _ _ _ w97 w109 _ _ _ _ _] -> w38
      tunnel: [w49 w57 w66 _ w96 w110 T7[] [{"AlliGator Q Event"=enum."Image:Image Histogram", "Data"=variant}, {"AlliGator Q Event"=enum."Image:Image Contrast", "Data"=variant}] ("AlliGator Actions") T7[] [{"AlliGator Q Event"=enum."Image:Image Histogram", "Data"=variant}, {"AlliGator Q Event"=enum."Image:Image Contrast", "Data"=variant}] ("AlliGator Actions") _ _ _] -> w36
      tunnel: w34 -> [w48 w58 _ _ w95 w106 _ _ _ _ _]
      tunnel: w35 -> [_ _ _ _ _ w105 _ _ _ _ _]
      tunnel: w33 -> [_ _ _ _ _ _ _ _ w139 w144 _]
      event "Image Histogram Active": Value Change {
        n20 = event-data() -> ("NewVal"=w52:bool)  [unwired: 1 in]
        n21 = case shown="True" w48 {
          tunnel: [_ w56] -> w49
          frame False {
          }
          frame True {
            n22 = Build Array(T7 {"AlliGator Q Event"=enum."Image:Image Histogram", "Data"=variant} ("element")) -> (w56:T7[])
          }
        }
        n23 = call "AlliGator Settings Storage.vi"("Get(F)/Set"=TRUE, "AlliGator Settings List"=AlliGator_Settings_List."Source Image:Image Histogram Active", "Variant Data in"=w52) -> ("Error Out"=w51:errorcluster)  [unwired: 7 in, 1 out]
      }
      event Value Change {
        n24 = event-data() -> ()  [unwired: 1 in, 1 out]
        n25 = case shown="True" w58 {
          tunnel: [_ w60] -> w57
          frame False {
          }
          frame True {
            n26 = Build Array(T7 {"AlliGator Q Event"=enum."Image:Image Histogram", "Data"=variant} ("element")) -> (w60:T7[])
          }
        }
      }
      event "Image Histogram": Cursor Move {
        w73 = T7 {"AlliGator Q Event"=enum."Image:Image Histogram Cursor Move", "Data"=variant} ("Time-Gated Phasor Q Element")
        n27 = event-data() -> ("Time"=w63:u32)  [unwired: 1 in]
        n28 = call "AlliGator Refnums Storage.vi"("AlliGator Refnum List"=AlliGator_Refnums_List."Dataset Ctrl Refnums") -> ("Error Out"=w70:errorcluster, "Data out"=w71:variant)  [unwired: 9 in]
        n29 = Variant To Data(error in=w70, type=T10 {"Current Data"=refnum, "Gate Image Slide"=refnum, "Time Point Slide"=refnum, "Current Time Stamp"=refnum, "Save Image"=refnum, "Displayed Image"=refnum, "Phasor Overlay Color"=refnum, "Image Color Scale"=refnum, "Use ROI as Search Area"=refnum, "Source Image ROI Color"=refnum, "True Pixel Value"=refnum, "Source Image Display"=refnum, "CPU"=refnum} ("Dataset Control References"), Variant=w71) -> (data=w68:T10, error out=w65:errorcluster)
        n30 = Unbundle By Name(w68) -> ("Source Image Display"=w67:refnum<vi>)
        n31 = property on="Auto-Adjust Contrast" class="Bool (strict)"() -> ("Value"=w62:bool)  [unwired: 2 in, 2 out]
        n32 = case shown="True" w62 {
          selector: w62 -> [_ w78]
          frame False {
          }
          frame True {
            n33 = Not(x=w78) -> (.not. x?=w77:bool)
            n34 = property on="Auto-Adjust Contrast" class="Bool (strict)"("Val(Sgnl)"=w77) -> ()  [unwired: 2 in, 2 out]
          }
        }
        n35 = call "AlliGator Filter Event.vi"("Error In"=w65, "Time"=w63, "AlliGatorr Q Element"=w73) -> ("Error Out"=w64:errorcluster, "Filter Event?"=w74:bool)  [unwired: 7 in]
        n36 = call "AlliGator Generic Image Display Mouse Move Flag.vi"("Image Control Refnum"=w67, "Read/Write"=Read-Write."Read") -> ("Flag (out)"=w75:bool)  [unwired: 7 in]
        n37 = Or(x=w74, y=w75) -> (x .or. y?=w76:bool)
        n38 = case shown="False" w76 {
          tunnel: w73 -> [w81 _]
          tunnel: [w80 _] -> w66
          tunnel: w67 -> [w79 _]
          frame False {
            # "event not filtered out"
            n39 = disable-structure shown="Disabled" {
              disable-tunnel: w79 -> [w82 _]
              frame Disabled {
                n40 = call "AlliGator Generic Image Display Mouse Move Flag.vi"("Image Control Refnum"=w82, "Flag (in)"=TRUE, "Read/Write"=Read-Write."Write") -> ()  [unwired: 6 in, 1 out]
              }
              frame Enabled {
              }
            }
            n41 = Build Array(w81) -> (w80:T7[])
          }
          frame True {
          }
        }
      }
      event "Image Histogram": Shortcut Menu Activation? {
        n42 = event-data() -> ("CtlRef"=w88:refnum<vi>, "MenuRef"=w87:refnum<k9>)  [unwired: 1 in]
        n43 = call "XY Graph Check-Uncheck Menu Items.vi"("Menu in"=w87, "XY Graph Refnum"=w88) -> ("Error Out (dup)"=w86:errorcluster, "Menu out"=w89:refnum<k9>, "XY Graph Refnum dup"=w90:T14)  [unwired: 6 in, 1 out]
        n44 = call "AlliGator Add Python Functions to Object Menu.vi"("error in (no error)"=w86, "Menu in"=w89, "Object Refnum"=w90) -> ("error out"=w85:errorcluster)  [unwired: 6 in, 2 out]
        n45 = event-data() -> ()  [unwired: 2 in, 1 out]
      }
      event "Image Histogram": Shortcut Menu Selection (User) {
        n46 = event-data() -> ("CtlRef"=w102:refnum<vi>, "Coords"=w101:T13, "ItemTag"=w100:string, "ItemPath"=w99:string)  [unwired: 1 in]
        n47 = call "AlliGator Keyboard ID.vi"() -> ("keys pressed"=w91:T15)  [unwired: 9 in, 2 out]
        n48 = Index Array(array=w91) -> (element=w93:T11)  [unwired: 1 in]
        n49 = Equal?(x=w93, y=T11."H" ("element")) -> (x = y?=w92:bool)
        n50 = Bundle By Name(cluster=T12 {"Item Tag"="", "XY Graph Refnum"=refnum, "Coords"={"Horizontal"=0, "Vertical"=0}, "Item Path"=""} ("XY Graph Event"), "XY Graph Refnum"=w102, "Coords"=w101, "Item Tag"=w100, "Item Path"=w99) -> (w103:T12)
        n51 = call "AlliGator Special Graph Menu Actions.vi"("Help?"=w92, "Animated Busy Icon"=w95, "XY Graph Event"=w103) -> ("Error Out"=w98:errorcluster, "Message"=w97:string, "AlliGator Actions"=w96:T7[])  [unwired: 6 in]
      }
      event "Use Image Histogram for Contrast": Value Change {
        n52 = event-data() -> ("CtlRef"=w107:refnum<vi>)  [unwired: 1 in]
        n53 = case shown="True" w106 {
          tunnel: w107 -> [_ w117]
          tunnel: w105 -> [_ w115]
          tunnel: [_ w114] -> w108
          tunnel: [_ T7[] [{"AlliGator Q Event"=enum."Image:Image Histogram", "Data"=variant}, {"AlliGator Q Event"=enum."Image:Image Contrast", "Data"=variant}] ("element")] -> w110
          tunnel: [_ w112] -> w109
          frame False {
          }
          frame True {
            n54 = property class="Bool (strict)"(reference=w117) -> (reference out=w116:refnum<vi>, error out=w118:errorcluster, "Label.Text"=w120:string, "Value"=w119:bool)  [unwired: 1 in]
            n55 = call "AlliGator Update Settings & Control.vi"("Error In"=w118, "Value"=w119, "Sender"=w115, "CtlRef"=w116) -> ("Error Out"=w111:errorcluster)  [unwired: 7 in]
            n56 = call "AlliGator Get Control Notebook String.vi"("error in (no error)"=w111, "Value"=w119, "Control Label"=w120) -> ("error out"=w114:errorcluster, "Notebook String"=w112:string)  [unwired: 7 in]
          }
        }
      }
      event "Auto-Adjust Contrast": Value Change {
        n57 = event-data() -> ("NewVal"=w122:bool)  [unwired: 1 in]
        n58 = call "AlliGator Settings Storage.vi"("Get(F)/Set"=TRUE, "AlliGator Settings List"=AlliGator_Settings_List."Source Image:Auto-Adjust Contrast", "Variant Data in"=w122) -> ()  [unwired: 7 in, 2 out]
      }
      event "Histogram Upper Percentile", "Histogram Lower Percentile": Value Change {
        n59 = event-data() -> ("CtlRef"=w128:refnum<vi>, "NewVal"=w127:dbl)  [unwired: 1 in]
        n60 = property class="DigNum (strict)"(reference=w128) -> ("Label.Text"=w129:string)  [unwired: 1 in, 2 out]
        n61 = case shown="\"Histogram Lower Percentile\"" w129 {
          tunnel: [_ w131 w135] -> w125
          tunnel: w127 -> [_ w130 w134]
          frame "", Default {
          }
          frame "Histogram Lower Percentile" {
            n62 = local write "Lower Percentile"(w130) -> ()
            n63 = call "AlliGator Settings Storage.vi"("Get(F)/Set"=TRUE, "AlliGator Settings List"=AlliGator_Settings_List."Source Image:Histogram Lower Percentile", "Variant Data in"=w130) -> ("Error Out"=w131:errorcluster)  [unwired: 7 in, 1 out]
          }
          frame "Histogram Upper Percentile" {
            n64 = local write "Upper Percentile"(w134) -> ()
            n65 = call "AlliGator Settings Storage.vi"("Get(F)/Set"=TRUE, "AlliGator Settings List"=AlliGator_Settings_List."Source Image:Histogram Upper Percentile", "Variant Data in"=w134) -> ("Error Out"=w135:errorcluster)  [unwired: 7 in, 1 out]
          }
        }
      }
      event Panel Close? {
        w138 = TRUE ("Pin Button")
        n66 = event-data() -> ()  [unwired: 1 in, 1 out]
        n67 = property on="Pin Button" class="Bool (strict)"("Value"=w138) -> (error out=w141:errorcluster)  [unwired: 2 in, 1 out]
        n68 = call "AlliGator Dock-Undock Subpanel Event.vi"("Error In"=w141, "Dock?"=w138, "VI in"=w139) -> ("Error Out"=w140:errorcluster)  [unwired: 8 in]
        n69 = event-data("Discard?"=w138) -> ()  [unwired: 1 in, 1 out]
      }
      event "Pin Button": Value Change {
        n70 = event-data() -> ("NewVal"=w143:bool)  [unwired: 1 in]
        n71 = call "AlliGator Dock-Undock Subpanel Event.vi"("Dock?"=w143, "VI in"=w144) -> ("Error Out"=w142:errorcluster)  [unwired: 9 in]
      }
      event User Event {
        n72 = event-data() -> ("subpanel"=w147:string, "event"=w146:string)  [unwired: 1 in]
        n73 = case shown="\"AlliGator\"" w147 {
          tunnel: w146 -> [_ w149]
          tunnel: [_ w148] -> w145
          frame "False", Default {
          }
          frame "AlliGator" {
            n74 = case shown="\"quit\"" w149 {
              tunnel: [_ TRUE] -> w148
              frame "False", Default {
              }
              frame "quit" {
              }
            }
          }
        }
      }
    }
    n75 = call "AlliGator Settings Storage.vi"("AlliGator Settings List"=AlliGator_Settings_List."Miscellaneous:Verbose Error Mode") -> ("Variant Data out"=w46:variant)  [unwired: 9 in, 1 out]
    n76 = call-poly "Variant to Data.vi"("Variant"=w46) -> ("Value"=w39:bool)  [unwired: 8 in]
    n77 = call "Send Message to Notebook.vi"("Error In"=w41, "Text"=w38, "Notebook Queue"=w40) -> ("Error Out"=w43:errorcluster, "Notebook Queue"=w42:refnum<queue>)  [unwired: 5 in]
    n78 = call "Light Theme Message Style.vi"() -> ()  [unwired: 1 out]
    n79 = call "AlliGator Queue Non Empty Events.vi"("Actions"=w36, "AlliGator Q"=w37) -> ()  [unwired: 9 in, 1 out]
    n80 = call "Send Error to Notebook.vi"("error in (no error)"=w43, "Verbose Error Messages (T)"=w39, "State Machine Case Error Source"="Image Histogram", "Notebook Q"=w42) -> ("Error Out"=w30:errorcluster)  [unwired: 7 in]
  }
  n81 = call "Tiny Clear Error.vi"("Error In"=w23) -> ("no Error Out"=w22:errorcluster)  [unwired: 8 in]
  n82 = Unregister For Events(event registration refnum=w24) -> (error out=w10:errorcluster)  [unwired: 1 in]
  n83 = invoke class="VI" method="FP.Close"(reference=w6, error in=w22) -> (error out=w11:errorcluster)  [unwired: 1 in, 2 out]
  n84 = Merge Errors(w11, w10) -> (w9:errorcluster)
  n85 = call "Tiny Clear Error.vi"("Error In"=w9) -> ()  [unwired: 8 in, 1 out]
